vi "Read Data Folder.vi"(8 "error in (no error)":errorcluster, 11 "Time Entry Store-INI in":refnum<class "Time Entry Store-INI.lvclass">) -> (0 "error out":errorcluster, 2 "Data Folder":path, 3 "Time Entry Store-INI out":refnum<class "Time Entry Store-INI.lvclass">)   [LabVIEW 2024, in "Time Entry Store-INI.lvclass"]
doc: "Reads one field of this class's private data. Generated by lvai_create_accessors from the class private data control."
uses:
  Time Entry Store-INI.lvclass
  Time Entry Store-INI.lvclass/Time Entry Store-INI.ctl
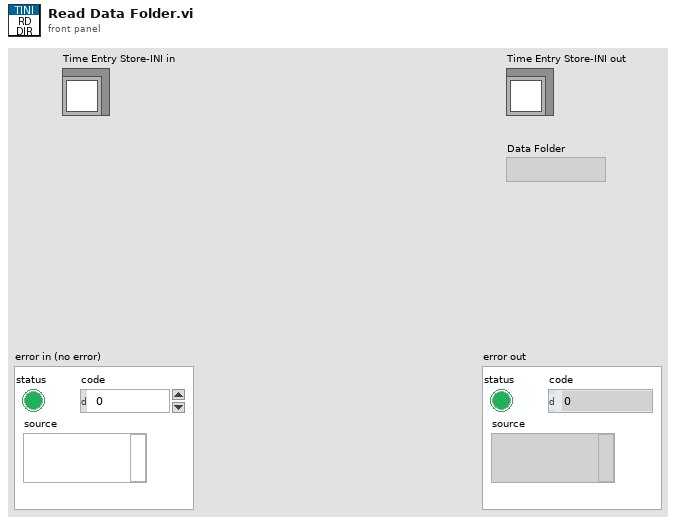
[diagram p1: front panel]
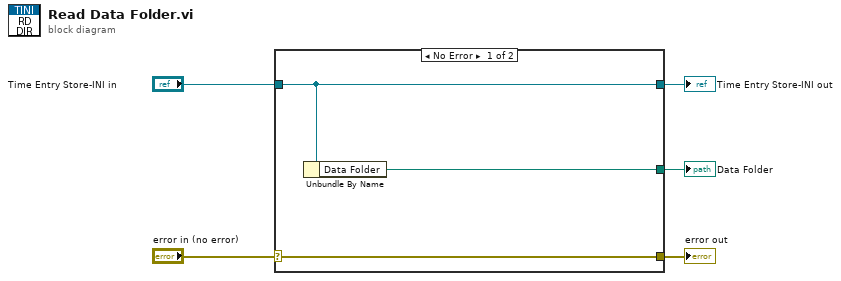
[diagram p0: block diagram]
diagram:
  n1 = case shown="No Error" "error in (no error)" {
    selector: "error in (no error)" -> [w8 w9]
    tunnel: [w8 w9] -> w4
    tunnel: [w7 w10] -> w2
    tunnel: "Time Entry Store-INI in" -> [w7 w10]
    tunnel: [w6 _] -> w1
    frame No Error {
      n2 = Unbundle By Name(w7) -> ("Data Folder"=w6:path)
    }
    frame Error {
    }
  }
  "error out" <- w4
  "Time Entry Store-INI out" <- w2
  "Data Folder" <- w1
